vi "Reverse (multiple).vi"(8 "error in (no error)":errorcluster, 11 "XY-data":cluster{"X-array":dbl[], "Y-array":dbl[]}[](array[cluster]) {"Y-array" format="%.2p"; "X-array" format="%.2p"}) -> (0 "error out":errorcluster, 3 "Reversed XY-data out":cluster{"X-array":dbl[], "Y-array":dbl[]}[](array[cluster]) {"Y-array" format="%.2p"; "X-array" format="%.2p"})   [LabVIEW 2019, in "xy_utilities.lvlib"]
doc: "Reverse both x and y arrays.\n\nWire data to the data input to determine the polymorphic instance to use or manually select the instance."
uses:
  xy_utilities.lvlib
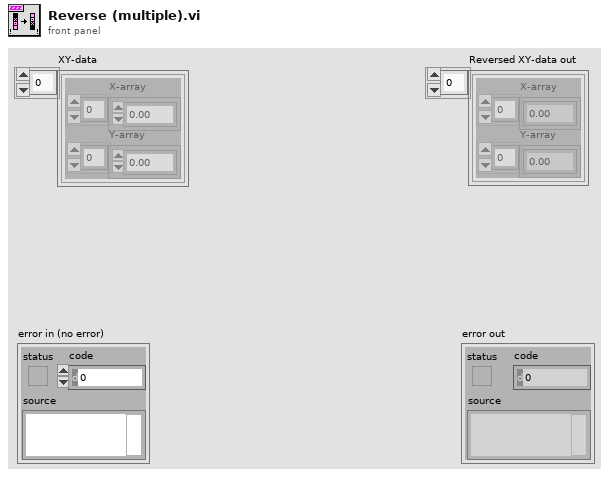
[diagram p1: front panel]
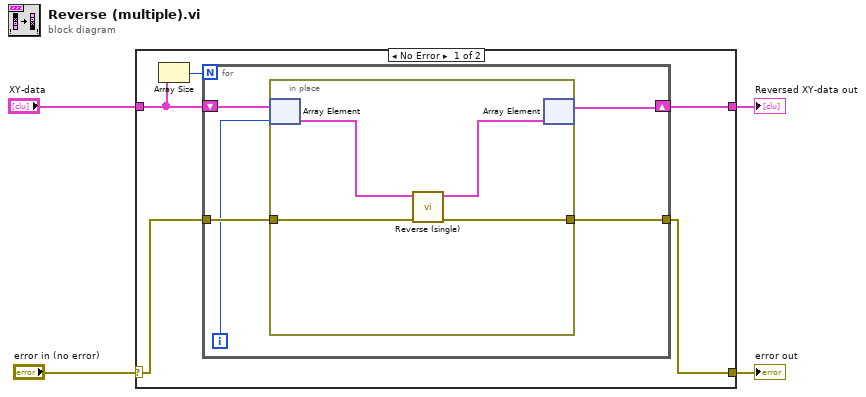
[diagram p0: block diagram]
diagram:
  n1 = case shown="No Error" "error in (no error)" {
    selector: "error in (no error)" -> [w7 w20]
    tunnel: [w8 w20] -> w3
    tunnel: "XY-data" -> [w5 w19]
    tunnel: [w9 w19] -> w1
    frame No Error {
      n2 = Array Size(array=w5) -> (size(s)=w6:i32)
      n3 = for {
        N: w6 -> [_]
        tunnel: w7 -> [w13]
        tunnel: [w14] -> w8
        shift-right: [w11] -> w9
        shift-left: w5 -> [w12]
        i -> [w10]
        n4 = in-place {
          in-place-border: [w18] -> w14
          in-place-border: w13 -> [w17]
          n5 = in-place-array #1(w12, w10) -> (w16:cluster{"X-array":dbl[], "Y-array":dbl[]})
          n6 = call "Reverse (single).vi"("error in (no error)"=w17, "XY-data"=w16) -> ("error out"=w18:errorcluster, "Reversed XY-data out"=w15:cluster{"X-array":dbl[], "Y-array":dbl[]})  [unwired: 8 in]
          n7 = in-place-array #1(w15) -> (w11:cluster{"X-array":dbl[], "Y-array":dbl[]}[])  [unwired: 1 out]
        }
      }
    }
    frame Error {
    }
  }
  "error out" <- w3
  "Reversed XY-data out" <- w1
